vi "Conversion_indice_chaine EPC.vi"(1 "Chaîne indice":string) -> (0 "Indice":i32)   [LabVIEW 2022 SP3]
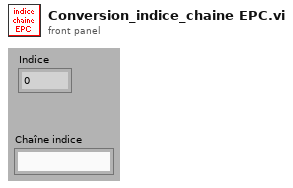
[diagram p1: front panel]
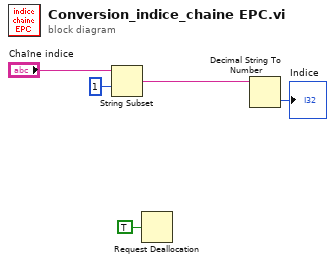
[diagram p0: block diagram]
diagram:
  n1 = String Subset(string="Chaîne indice", offset (0)=1) -> (substring=w1:string)  [unwired: 1 in]
  n2 = Request Deallocation(TRUE ("flag")) -> ()
  n3 = Decimal String To Number(string=w1) -> (number=→"Indice":i32)  [unwired: 2 in, 1 out]
